vi "TestMulticolumnListboxAccess.vi"(8 "error in":errorcluster) -> (0 "error out":errorcluster)   [LabVIEW 2016, in "WeatherReportTests.lvlib"]
uses:
  WeatherReportTests.lvlib
  APIs/Stimulus/ControlValue/Controls/MC Listbox/SetValueByItemName.vi
  APIs/Assert/AssertControlValue/Equal.vi
  APIs/Stimulus/VI/CloseVI.vi
  <vilib>/addons/_JKI Toolkits/Caraya/classes/Test/Test.lvclass
  Drona.lvlib
  APIs/Assert/AssertControlValue/AssertControlValue.lvlib
  APIs/Stimulus/VI/VI.lvlib
  APIs/Stimulus/ControlValue/Controls/MC Listbox/StimulusMCListbox.lvlib
panel:
  # "Drona Test Multicolumn Access"
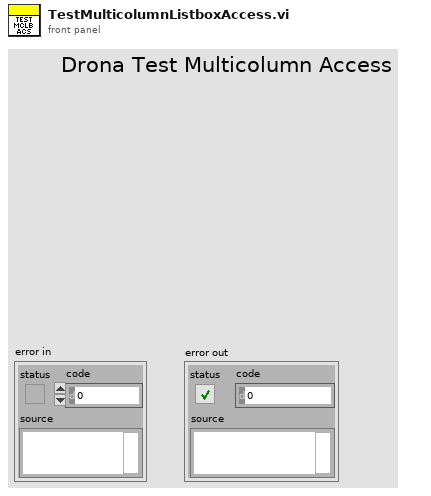
[diagram p1: front panel]
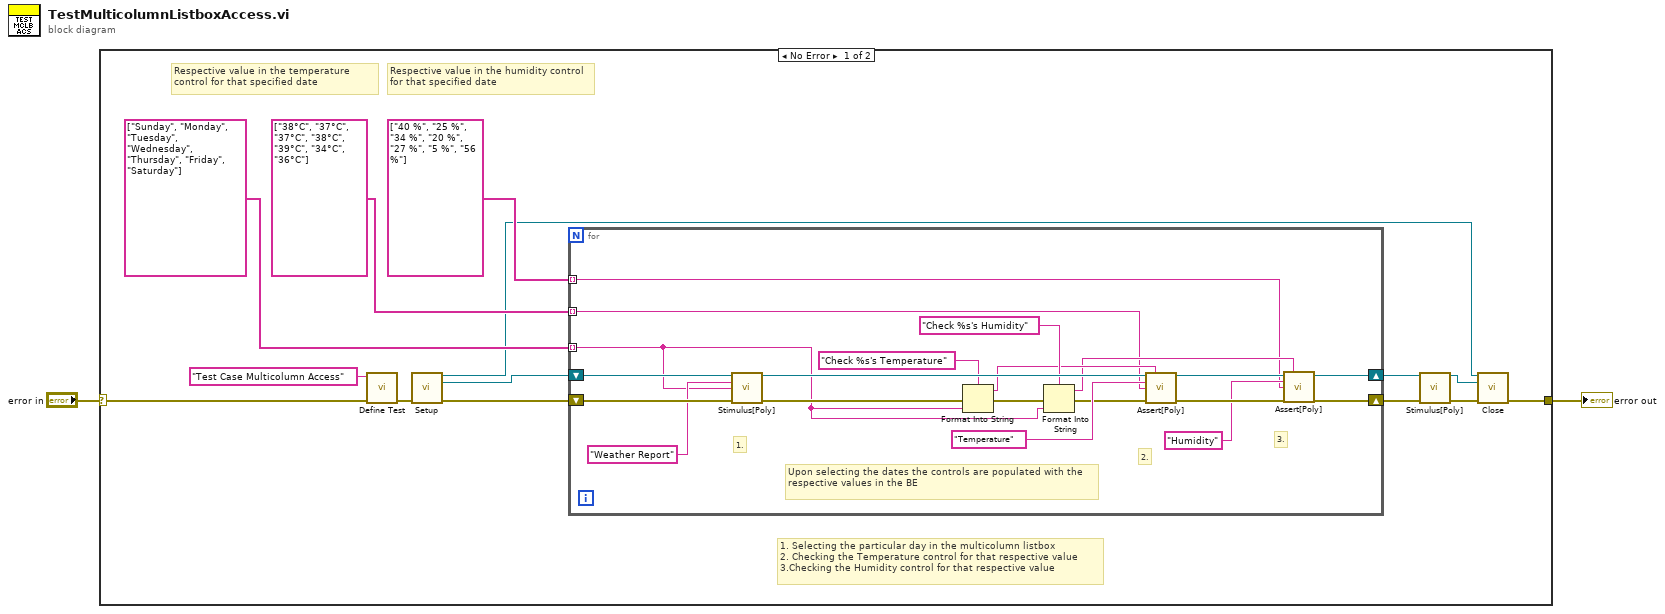
[diagram p0: block diagram]
diagram:
  n1 = case shown="No Error" "error in" {
    selector: "error in" -> [w16 w37]
    tunnel: [w11 w37] -> w1
    frame No Error {
      # "1. Selecting the particular day in the multicolumn listbox\n2. Checking the Temperature control for that respective value\n3.Checking the Humidity control for that respective value"
      # "Respective value in the humidity control for that specified date"
      # "Respective value in the temperature control for that specified date"
      n2 = call <vilib>:"Define Test.vi"("error in (no error)"=w16, "Label (VI Title)"="Test Case Multicolumn Access") -> ("error out"=w14:errorcluster)  [unwired: 8 in, 1 out]
      n3 = call "Setup.vi"("error in"=w14) -> ("Application Ref"=w3:refnum<vi>, "VI Reference Out"=w13:refnum<vi>, "error out"=w12:errorcluster)  [unwired: 12 in]
      n4 = for {
        shift-right: [w30] -> w7
        shift-left: w13 -> [w36]
        shift-right: [w31] -> w8
        shift-left: w12 -> [w35]
        tunnel: string[] ["Sunday", "Monday", "Tuesday", "Wednesday", "Thursday", "Friday", "Saturday"] ("Item Name") -> [w19] mode=indexing
        tunnel: string[] ["38°C", "37°C", "37°C", "38°C", "39°C", "34°C", "36°C"] ("Control Path") -> [w17] mode=indexing
        tunnel: string[] ["40 %", "25 %", "34 %", "20 %", "27 %", "5 %", "56 %"] ("Control Path") -> [w18] mode=indexing
        # "Upon selecting the dates the controls are populated with the respective values in the BE"
        # "3."
        # "2."
        # "1."
        n5 = call-poly "Stimulus[Poly].vi"("VI Reference In"=w36, "Control Path"="Weather Report", "Item Name"=w19, "Error In"=w35) -> ("VI Reference Out"=w33:refnum<vi>, "Error Out"=w32:errorcluster)  [unwired: 10 in]
        n6 = Format Into String(format string="Check %s's Temperature", error in=w32, w19) -> (resulting string=w21:string, error out=w23:errorcluster)  [unwired: 1 in]
        n7 = Format Into String(format string="Check %s's Humidity", error in=w23, w19) -> (resulting string=w20:string, error out=w22:errorcluster)  [unwired: 1 in]
        n8 = call-poly "Assert[Poly].vi"("VI Reference In"=w33, "Test Label"=w21, "Control Path"="Temperature", "Control Value"=w17, "Error In"=w22) -> ("VI Reference Out"=w27:refnum<vi>, "Error Out"=w28:errorcluster)  [unwired: 8 in, 1 out]
        n9 = call-poly "Assert[Poly].vi"("VI Reference In"=w27, "Test Label"=w20, "Control Path"="Humidity", "Control Value"=w18, "Error In"=w28) -> ("VI Reference Out"=w30:refnum<vi>, "Error Out"=w31:errorcluster)  [unwired: 8 in, 1 out]
      }
      n10 = call-poly "Stimulus[Poly].vi"("VI Reference In"=w7, "error in"=w8) -> ("VI Reference Out"=w9:refnum<vi>, "error out"=w10:errorcluster)  [unwired: 12 in]
      n11 = call "Close.vi"("Application Ref"=w3, "VI Reference"=w9, "error in"=w10) -> ("error out"=w11:errorcluster)  [unwired: 12 in]
    }
    frame Error {
    }
  }
  "error out" <- w1
